vi "Execution Engine.vi"(11 "System":refnum<class "bt_System.lvclass">) -> ()   [LabVIEW 2021, in "BT.lvlib" / "bt_System.lvclass"]
uses:
  bt_System.lvclass
  Support/Nodes/abs_Node/Status.ctl
  bt_System.lvclass/bt_System.ctl
  Support/Nodes/abs_Node/bt_Node.lvclass
panel:
  out "Status":T1
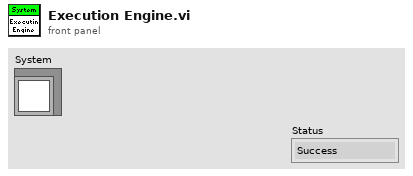
[diagram p1: front panel]
types:
  T1 = typedef "BT.lvlib/bt_Node.lvclass/Status.ctl" = enum16{"Success", "Failure", "Running"}
  T2 = typedef "Rendezvous RefNum" = refnum<k1>
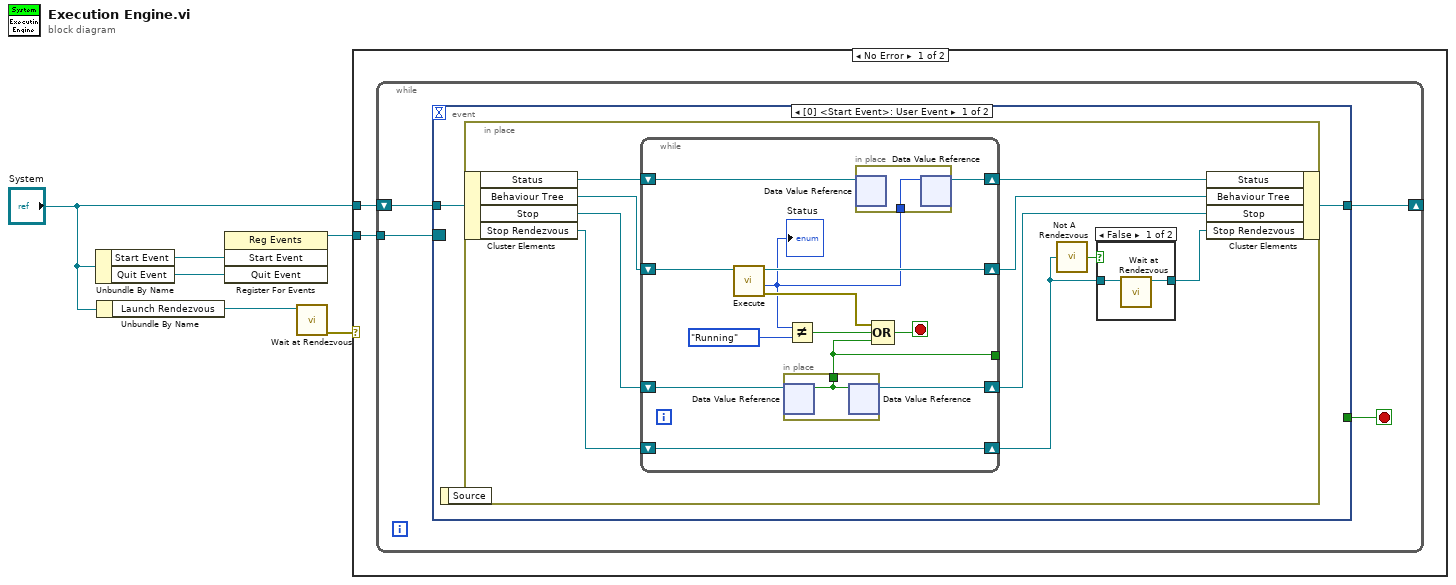
[diagram p0: block diagram]
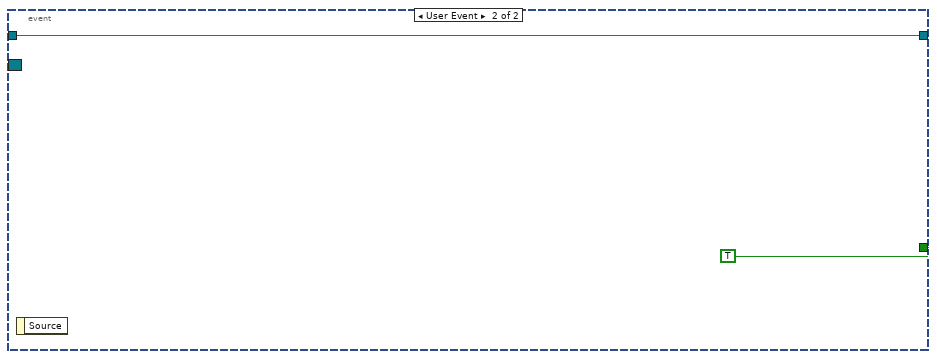
[diagram p3: hidden frame]
diagram:
  n1 = Unbundle By Name("System") -> ("Start Event"=w3:refnum<user-event>, "Quit Event"=w2:refnum<user-event>)
  n2 = Unbundle By Name("System") -> ("Launch Rendezvous"=w6:T2)
  n3 = register-events(w3, w2) -> (reference out=w5:refnum<event-registration>)  [unwired: 2 in, 1 out]
  n4 = call <vilib>:"Wait at Rendezvous.vi"("rendezvous"=w6) -> ("error out"=w1:errorcluster)  [unwired: 4 in, 2 out]
  n5 = case shown="No Error" w1 {
    tunnel: w5 -> [w8 _]
    tunnel: "System" -> [w7 _]
    frame No Error {
      n6 = while {
        tunnel: w8 -> [w12]
        shift-right: [w10] -> _
        shift-left: w7 -> [w11]
        stop <- w9 stop-if-true
        n7 = event shown="[0] <Start Event>: User Event" {
          selector: w12 -> [_ _]
          dyn-events: _ -> [_ _]
          timeout: _ -> [_ _]
          tunnel: w11 -> [w14 w44]
          tunnel: [w13 w44] -> w10
          tunnel: [_ TRUE] -> w9
          event User Event {
            n8 = event-data() -> ()  [unwired: 1 in, 1 out]
            n9 = in-place {
              n10 = in-place-cluster #1(w14) -> ("Status"=w24:refnum<data-value>, "Behaviour Tree"=w23:refnum<class "bt_Node.lvclass">, "Stop"=w20:refnum<data-value>, "Stop Rendezvous"=w18:T2)
              n11 = while {
                shift-right: [w37] -> w22
                shift-left: w23 -> [w38]
                shift-right: [w32] -> w19
                shift-left: w20 -> [w33]
                shift-right: [w29] -> w21
                shift-left: w24 -> [w30]
                tunnel: [w31] -> _
                shift-right: [w36] -> w16
                shift-left: w18 -> [w36]
                stop <- w40 stop-if-true
                n12 = call-dynamic "Execute.vi"("Node in"=w38) -> ("error out"=w39:errorcluster, "Status"=w28:T1, "Node out"=w37:refnum<class "bt_Node.lvclass">)  [unwired: 8 in]
                "Status" <- w28
                n13 = in-place {
                  in-place-border: [w42] -> w31
                  n14 = in-place-dvr #2(w33) -> (w42:bool)  [unwired: 1 out]
                  n15 = in-place-dvr #2(w42) -> (w32:refnum<data-value>)  [unwired: 1 out]
                }
                n16 = Not Equal?(x=w28, y=Status."Running") -> (x != y?=w35:bool)
                n17 = in-place {
                  in-place-border: w28 -> [w41]
                  n18 = in-place-dvr #3(w30) -> ()  [unwired: 2 out]
                  n19 = in-place-dvr #3(w41) -> (w29:refnum<data-value>)  [unwired: 1 out]
                }
                n20 = Compound Arithmetic op=OR(w39, w35, w31) -> (w40:bool)
              }
              n21 = call <vilib>:"Not A Rendezvous.vi"("rendezvous"=w16) -> ("not a rendezvous"=w15:bool)
              n22 = case shown="False" w15 {
                tunnel: w16 -> [w26 w27]
                tunnel: [w25 w27] -> w17
                frame False {
                  n23 = call <vilib>:"Wait at Rendezvous.vi"("rendezvous"=w26) -> ("rendezvous out"=w25:T2)  [unwired: 4 in, 2 out]
                }
                frame True {
                }
              }
              n24 = in-place-cluster #1("Status"=w21, "Behaviour Tree"=w22, "Stop"=w19, "Stop Rendezvous"=w17) -> (w13:refnum<class "bt_System.lvclass">)
            }
          }
          event User Event {
            n25 = event-data() -> ()  [unwired: 1 in, 1 out]
          }
        }
      }
    }
    frame Error {
    }
  }
